vi "Evaluate Row.vi"(6 "Headers":string[](array[string]), 9 "Comparators":T1(array[cluster]), 10 "Boolean Connectors":string[](array[string]), 11 "Row":string[](array[string])) -> (3 "Match?":bool)   [LabVIEW 2025, in "CAN-LIN Raw Bus Capture UI.lvlib"]
uses:
  CAN-LIN Raw Bus Capture UI.lvlib
  Table_Filtering/Table_Filtering.lvlib
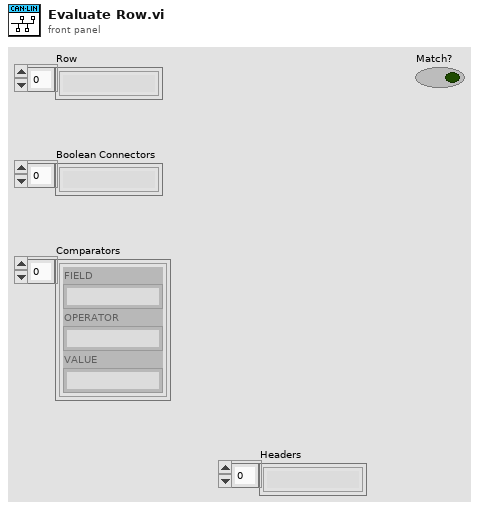
[diagram p1: front panel]
types:
  T1 = cluster{"FIELD":string, "OPERATOR":string, "VALUE":string}[]
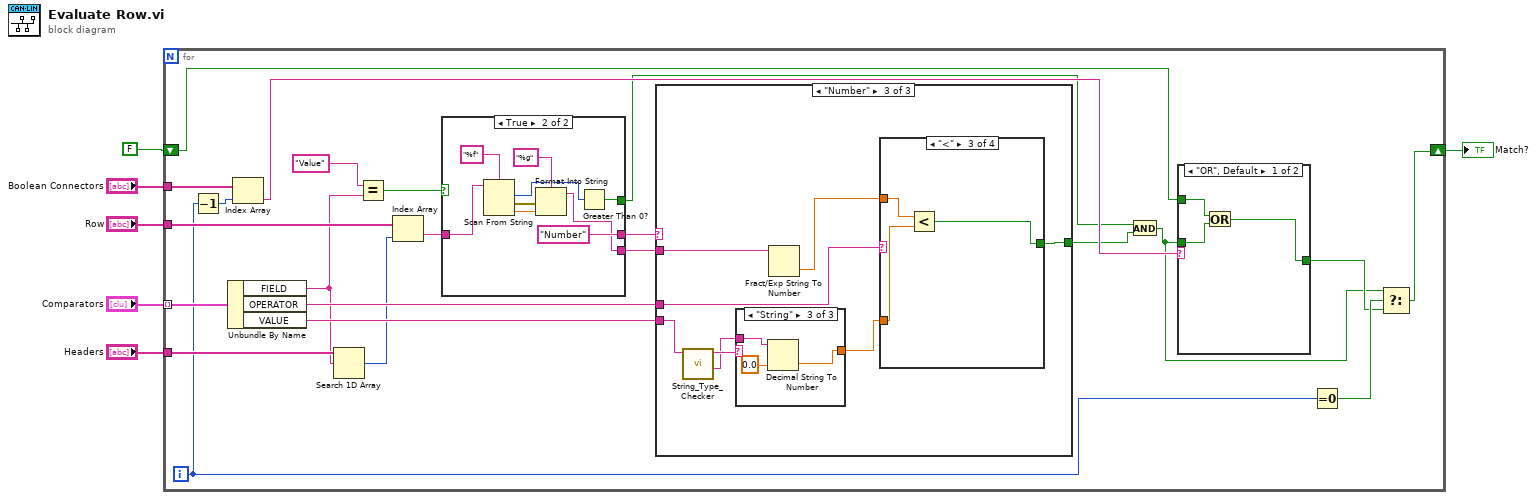
[diagram p0: block diagram]
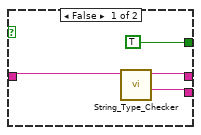
[diagram p2: hidden frame]
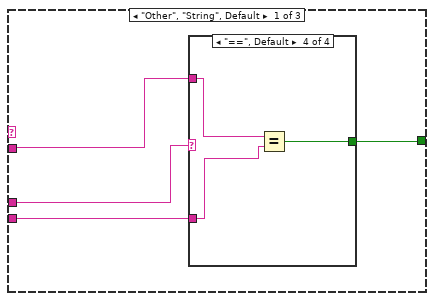
[diagram p3: hidden frame]
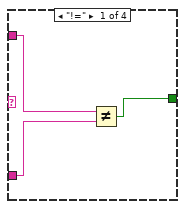
[diagram p4: hidden frame]
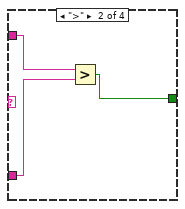
[diagram p5: hidden frame]
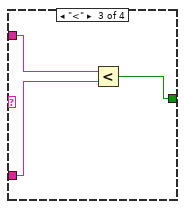
[diagram p6: hidden frame]
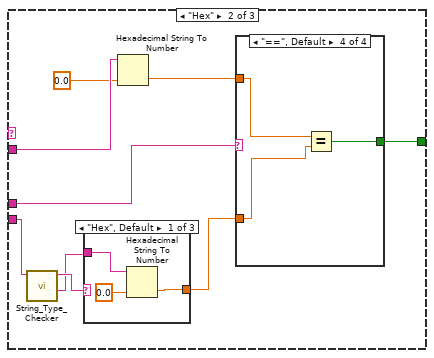
[diagram p7: hidden frame]
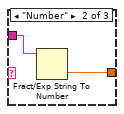
[diagram p8: hidden frame]
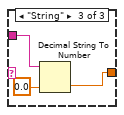
[diagram p9: hidden frame]
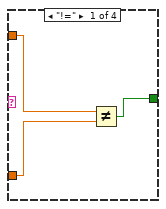
[diagram p10: hidden frame]
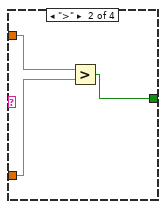
[diagram p11: hidden frame]
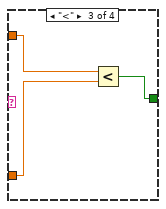
[diagram p12: hidden frame]
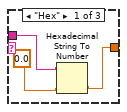
[diagram p13: hidden frame]
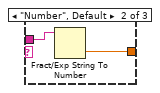
[diagram p14: hidden frame]
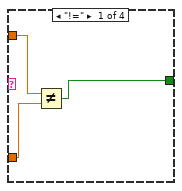
[diagram p15: hidden frame]
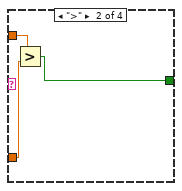
[diagram p16: hidden frame]
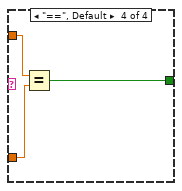
[diagram p17: hidden frame]
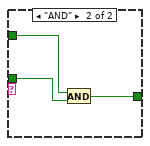
[diagram p18: hidden frame]
diagram:
  n1 = for {
    tunnel: "Headers" -> [w28]
    tunnel: "Comparators" -> [w29] mode=indexing
    shift-right: [w13] -> w6
    shift-left: FALSE -> [w25]
    tunnel: "Boolean Connectors" -> [w27]
    tunnel: "Row" -> [w18]
    i -> [w16]
    n2 = Decrement(x=w16) -> (x-1=w26:i32)
    n3 = Unbundle By Name(w29) -> ("FIELD"=w12:string, "OPERATOR"=w23:string, "VALUE"=w24:string)
    n4 = Index Array(array=w27, index=w26) -> (element=w22:string)
    n5 = Search 1D Array(1D array=w28, element=w12) -> (index of element=w21:i32)  [unwired: 1 in]
    n6 = Equal?(x="Value", y=w12) -> (x = y?=w10:bool)
    n7 = Index Array(array=w18, index=w21) -> (element=w17:string)
    n8 = case shown="True" w10 {
      tunnel: [w33 "Number" ("Type")] -> w20
      tunnel: [w32 w34] -> w19
      tunnel: w17 -> [w31 w37]
      tunnel: [TRUE w36] -> w9
      frame False {
        n9 = call "String_Type_Checker.vi"("String"=w31) -> ("Number"=w32:string, "Type"=w33:string)  [unwired: 9 in]
      }
      frame True {
        n10 = Scan From String(format string="%f", input string=w37) -> (offset past scan=w35:u32, error out=w41:errorcluster, output 1=w40:dbl)  [unwired: 3 in, 1 out]
        n11 = Format Into String(format string="%g", error in=w41, w40) -> (resulting string=w34:string)  [unwired: 1 in, 1 out]
        n12 = Greater Than 0?(x=w35) -> (x > 0?=w36:bool)
      }
    }
    n13 = case shown="\"Number\"" w20 {
      tunnel: w19 -> [w46 w67 w95]
      tunnel: w24 -> [w43 w62 w91]
      tunnel: w23 -> [w45 w65 w94]
      tunnel: [w44 w64 w93] -> w8
      frame "Other", "String", Default {
        n14 = case shown="\"==\", Default" w45 {
          tunnel: w46 -> [w48 w52 w55 w56]
          tunnel: w43 -> [w47 w51 w54 w58]
          tunnel: [w49 w50 w53 w57] -> w44
          frame "!=" {
            n15 = Not Equal?(x=w48, y=w47) -> (x != y?=w49:bool)
          }
          frame ">" {
            n16 = Greater?(x=w52, y=w51) -> (0:w50:bool)
          }
          frame "<" {
            n17 = Less?(x=w55, y=w54) -> (x < y?=w53:bool)
          }
          frame "==", Default {
            n18 = Equal?(x=w56, y=w58) -> (x = y?=w57:bool)
          }
        }
      }
      frame "Hex" {
        n19 = call "String_Type_Checker.vi"("String"=w62) -> ("Number"=w59:string, "Type"=w60:string)  [unwired: 9 in]
        n20 = case shown="\"Hex\", Default" w60 {
          tunnel: [w68 w72 w75] -> w63
          tunnel: w59 -> [w70 w71 w73]
          frame "Hex", Default {
            n21 = Hexadecimal String To Number(string=w70, default (0uL)=0.0) -> (number=w68:dbl)  [unwired: 1 in, 1 out]
          }
          frame "Number" {
            n22 = Fract/Exp String To Number(string=w71) -> (number=w72:dbl)  [unwired: 3 in, 1 out]
          }
          frame "String" {
            n23 = Decimal String To Number(string=w73, default (0L)=0.0) -> (number=w75:dbl)  [unwired: 1 in, 1 out]
          }
        }
        n24 = Hexadecimal String To Number(string=w67, default (0uL)=0.0) -> (number=w66:dbl)  [unwired: 1 in, 1 out]
        n25 = case shown="\"==\", Default" w65 {
          tunnel: w66 -> [w77 w81 w84 w85]
          tunnel: w63 -> [w76 w80 w83 w87]
          tunnel: [w78 w79 w82 w86] -> w64
          frame "!=" {
            n26 = Not Equal?(x=w77, y=w76) -> (x != y?=w78:bool)
          }
          frame ">" {
            n27 = Greater?(x=w81, y=w80) -> (0:w79:bool)
          }
          frame "<" {
            n28 = Less?(x=w84, y=w83) -> (x < y?=w82:bool)
          }
          frame "==", Default {
            n29 = Equal?(x=w85, y=w87) -> (x = y?=w86:bool)
          }
        }
      }
      frame "Number" {
        n30 = call "String_Type_Checker.vi"("String"=w91) -> ("Number"=w89:string, "Type"=w90:string)  [unwired: 9 in]
        n31 = case shown="\"String\"" w90 {
          tunnel: [w96 w100 w103] -> w88
          tunnel: w89 -> [w98 w99 w101]
          frame "Hex" {
            n32 = Hexadecimal String To Number(string=w98, default (0uL)=0.0) -> (number=w96:dbl)  [unwired: 1 in, 1 out]
          }
          frame "Number", Default {
            n33 = Fract/Exp String To Number(string=w99) -> (number=w100:dbl)  [unwired: 3 in, 1 out]
          }
          frame "String" {
            n34 = Decimal String To Number(string=w101, default (0L)=0.0) -> (number=w103:dbl)  [unwired: 1 in, 1 out]
          }
        }
        n35 = Fract/Exp String To Number(string=w95) -> (number=w92:dbl)  [unwired: 3 in, 1 out]
        n36 = case shown="\"<\"" w94 {
          tunnel: w88 -> [w105 w109 w112 w115]
          tunnel: [w106 w108 w111 w114] -> w93
          tunnel: w92 -> [w104 w107 w110 w113]
          frame "!=" {
            n37 = Not Equal?(x=w104, y=w105) -> (x != y?=w106:bool)
          }
          frame ">" {
            n38 = Greater?(x=w107, y=w109) -> (0:w108:bool)
          }
          frame "<" {
            n39 = Less?(x=w110, y=w112) -> (x < y?=w111:bool)
          }
          frame "==", Default {
            n40 = Equal?(x=w113, y=w115) -> (x = y?=w114:bool)
          }
        }
      }
    }
    n41 = And(x=w9, y=w8) -> (x .and. y?=w7:bool)
    n42 = case shown="\"OR\", Default" w22 {
      tunnel: w25 -> [w117 w121]
      tunnel: [w118 w120] -> w14
      tunnel: w7 -> [w116 w119]
      frame "OR", Default {
        n43 = Or(x=w117, y=w116) -> (x .or. y?=w118:bool)
      }
      frame "AND" {
        n44 = And(x=w121, y=w119) -> (x .and. y?=w120:bool)
      }
    }
    n45 = Equal To 0?(x=w16) -> (x = 0?=w15:bool)
    n46 = Select(t=w7, s=w15, f=w14) -> (s? t:f=w13:bool)
  }
  "Match?" <- w6
